vi "to string.vi"(8 "error in":errorcluster, 11 "SystemLin Tag Module configuration in":refnum<class "SystemLink configuration.lvclass">) -> (0 "error out":errorcluster, 1 "data":string, 2 "version":string, 3 "SystemLin Tag Module configuration out":refnum<class "SystemLink configuration.lvclass">)   [LabVIEW 2015, in "SystemLink configuration.lvclass"]
doc: "Provides an interface for saving a module configuration to a file or other serialized data source. It is recommended that all children of this class store data in two sets--data required for its own initialization, and any data required for parent initialization--and that each implementation uses the <b>Call Parent Method</b> primitive to serialize parent information."
uses:
  SystemLink configuration.lvclass
  SystemLink configuration.lvclass/SystemLink configuration.ctl
  current version.vi
  <vilib>/NI/Tag Bus Module Framework/module configuration/TBM module configuration.lvclass
  <vilib>/NI/Tag Bus Module Framework/channel/TBM channel.lvclass
  <vilib>/NI/Configuration Framework/serializable configuration/NISE_CEF_serializable configuration.lvclass
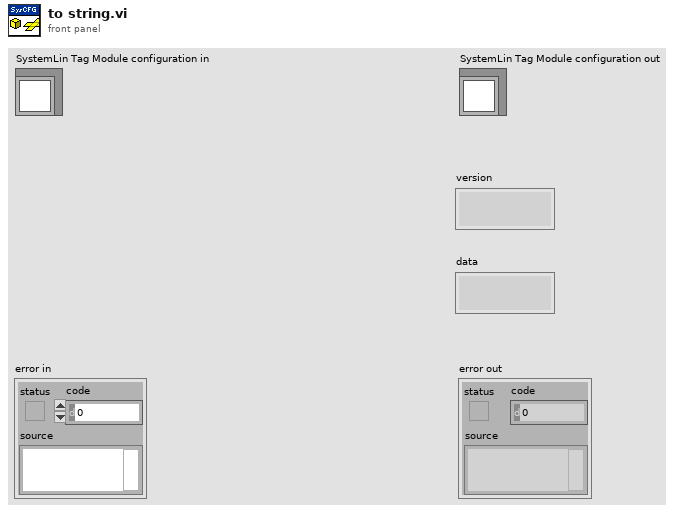
[diagram p1: front panel]
types:
  T1 = typedef "SystemLink configuration.lvclass/Line.ctl" = cluster{"channel":refnum<class "TBM channel.lvclass">, "Data Tag Type":T2}
  T2 = typedef "SystemLink configuration.lvclass/Data Tag Type.ctl" = enum16{"Double", "Single", "I32", "I16", "I8", "U64", "U32", "U16", "U8", "Boolean", "String", "Timestamp"}
  T3 = typedef "SystemLink configuration.lvclass/Connection Configuration.ctl" = cluster{"Connection Type":T4, "AMQP":cluster{"Configuration ID":string}, "HTTP":cluster{"Verify Server?":bool, "Server URL":string, "CA Certificate File":string, "User Info":cluster{"Username":string, "Password":string}, "API Key":string}}
  T4 = typedef "SystemLink configuration.lvclass/Connection Type.ctl" = enum16{"AMQP", "HTTP", "API Key (SystemLink Cloud)"}
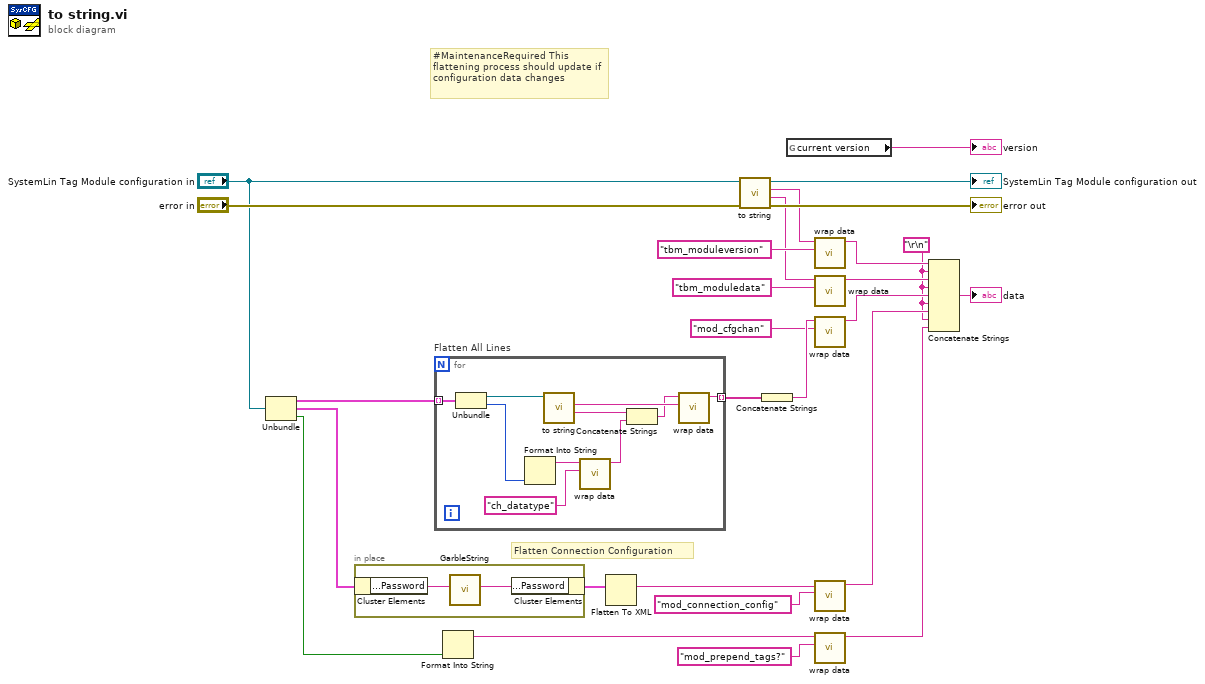
[diagram p0: block diagram]
diagram:
  w4 = "\r\n"
  # "Flatten Connection Configuration"
  # "#MaintenanceRequired This flattening process should update if configuration data changes"
  n1 = Unbundle("SystemLin Tag Module configuration in") -> (w14:T1[], w7:T3, w5:bool)
  n2 = in-place {
    n3 = in-place-cluster #1(w7) -> ("HTTP.User Info.Password"=w29:string)
    n4 = call "GarbleString.vi"("String In"=w29) -> ("String Out"=w28:string)  [unwired: 10 in]
    n5 = in-place-cluster #1("HTTP.User Info.Password"=w28) -> (w6:T3)
  }
  n6 = for "Flatten All Lines" {
    tunnel: w14 -> [w39] mode=indexing
    tunnel: [w32] -> w13 mode=indexing
    n7 = Unbundle(w39) -> ("channel"=w38:refnum<class "TBM channel.lvclass">, "Data Tag Type"=w35:T2)
    n8 = Format Into String(w35) -> (resulting string=w34:string)  [unwired: 3 in, 1 out]
    n9 = call-dynamic "to string.vi"("channel in"=w38) -> ("channel data"=w36:string, "identifier"=w37:string)  [unwired: 7 in, 2 out]
    n10 = call <vilib>:"wrap data.vi"("identifier"="ch_datatype", "data to wrap"=w34) -> ("wrapped data"=w30:string)  [unwired: 9 in]
    n11 = Concatenate Strings(w36, w30) -> (w31:string)
    n12 = call <vilib>:"wrap data.vi"("identifier"=w37, "data to wrap"=w31) -> ("wrapped data"=w32:string)  [unwired: 9 in]
  }
  n13 = Format Into String(w5) -> (resulting string=w2:string)  [unwired: 3 in, 1 out]
  n14 = Flatten To XML(anything=w6) -> (xml string=w10:string)
  n15 = call-parent "to string.vi"("error in"="error in", "module configuration in"="SystemLin Tag Module configuration in") -> ("error out"=→"error out":errorcluster, "data"=w18:string, "version"=w19:string, "module configuration out"=→"SystemLin Tag Module configuration out":refnum<class "SystemLink configuration.lvclass">)  [unwired: 6 in]
  n16 = Concatenate Strings(w13) -> (w12:string)
  n17 = global read "current version.vi" "current version"() -> (→"version":string)
  n18 = call <vilib>:"wrap data.vi"("identifier"="tbm_moduleversion" ("additional identifier"), "data to wrap"=w19) -> ("wrapped data"=w21:string)  [unwired: 9 in]
  n19 = call <vilib>:"wrap data.vi"("identifier"="tbm_moduledata" ("additional identifier"), "data to wrap"=w18) -> ("wrapped data"=w20:string)  [unwired: 9 in]
  n20 = call <vilib>:"wrap data.vi"("identifier"="mod_cfgchan", "data to wrap"=w12) -> ("wrapped data"=w15:string)  [unwired: 9 in]
  n21 = call <vilib>:"wrap data.vi"("identifier"="mod_connection_config", "data to wrap"=w10) -> ("wrapped data"=w9:string)  [unwired: 9 in]
  n22 = call <vilib>:"wrap data.vi"("identifier"="mod_prepend_tags?", "data to wrap"=w2) -> ("wrapped data"=w1:string)  [unwired: 9 in]
  n23 = Concatenate Strings(w21, w4, w20, w4, w15, w4, w9, w4, w1) -> (→"data":string)
